vi "Some_Code.vi"() -> ()   [LabVIEW 2026]
panel:
  out "Tank":dbl(slide) scale=0.0..10.0
  out "error out":errorcluster
  in  "error in (no error)":errorcluster
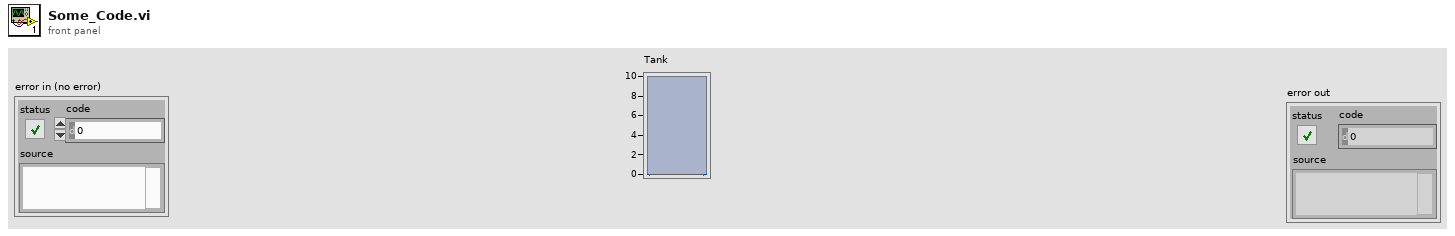
[diagram p1: front panel]
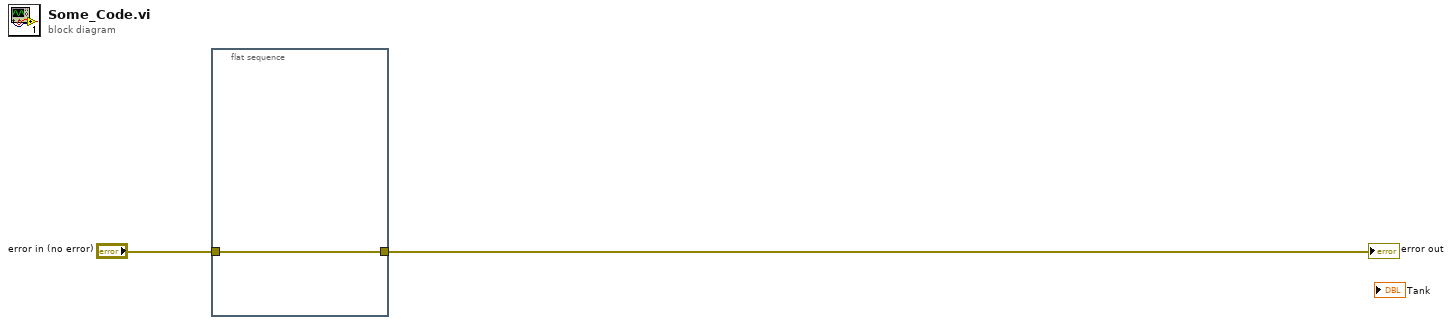
[diagram p0: block diagram]
diagram:
  n1 = flat-sequence {
    tunnel: "error in (no error)" -> [w3]
    tunnel: [w3] -> w1
    frame #0 {
    }
  }
  "error out" <- w1
